vi "Create Property.vi"(8 "error in":errorcluster, 10 "Labview Type":T1, 11 "Description":string) -> (0 "error out":errorcluster, 3 "JSON Schema Property out":string)   [LabVIEW 2020, in "JSON Schema Generator.lvlib"]
uses:
  JSON Schema Generator.lvlib
  <vilib>/Utility/Data Type/Type Definitions/Data Type.ctl
  aea4ecb6-ee08-4fcf-bd9c-6a72ca557f06.vi
  1a4a9289-16be-4b5e-ac83-e746006c8e55.vi
  <vilib>/JDP Science/JSONtext/Variant to JSON Text.vi
  <vilib>/JDP Science/JSONtext/Get all Object Items.vi
  <vilib>/JDP Science/JSONtext/Set Multiple Object Items.vi
  <vilib>/JDP Science/JSONtext/LVClass Serializer/JSONtext LVClass Serializer.lvclass
  <vilib>/JDP Science/JSONtext/JSONtext.lvlib
  <vilib>/Utility/Data Type/NI_Data Type.lvlib
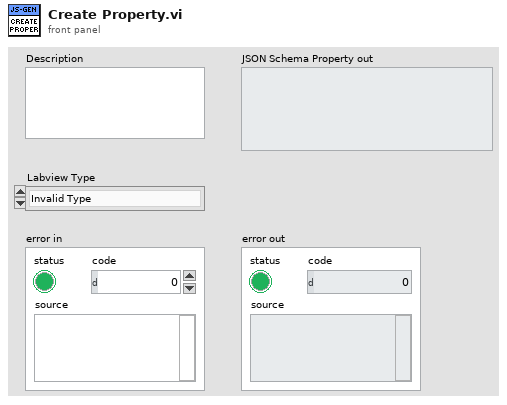
[diagram p1: front panel]
types:
  T1 = typedef "NI_Data Type.lvlib/Data Type.ctl" = enum8{"Invalid Type", "Void", "I8", "I16", "I32", "I64", "U8", "U16", "U32", "U64", "Single Float", "Double Float", "Extended Float", "Single Complex", "Double Complex", "Extended Complex", "Enum U8", "Enum U16", "Enum U32", "Enum U64", "Single Float With Unit", "Double Float With Unit", "Extended Float With Unit", "Single Complex with Unit", "Double Complex with Unit", "Extended Complex with Unit", "Boolean", "String", "Path", "Picture", "Tag", "Array", "Cluster", "Variant", "LV Variant", "Waveform", "Timestamp", "Digital Waveform", "Digital Data", "ExpressData", "Refnum", "External Data", "VI", "Poly VI", "LabVIEW Class Instance", "Fixed Point", "Set Collection", "Map Collection"}
  T2 = typedef "JSONtext.lvlib/JSON Value Type.ctl" = enum16{"Not a JSON Value", "JSON Object", "JSON Array", "String", "Number", "true", "false", "null"}
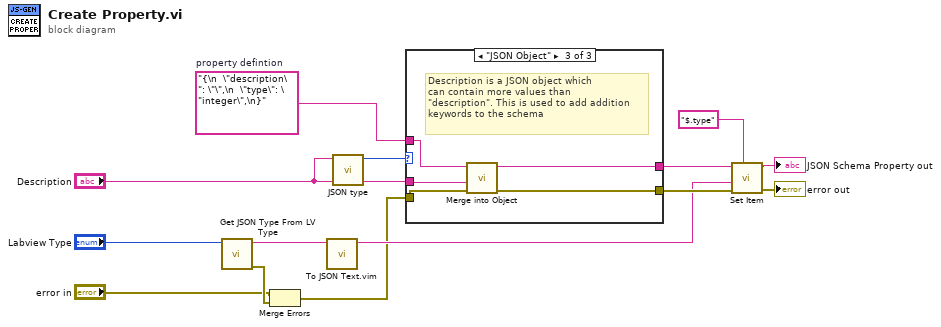
[diagram p0: block diagram]
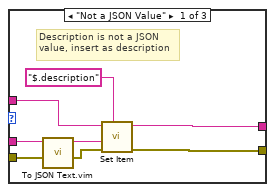
[diagram p2: hidden frame]
diagram:
  w11 = "{\n  \"description\": \"\",\n  \"type\": \"integer\",\n}"  # property defintion
  n1 = call "Get JSON Type From LV Type.vi"("Labview Datatype"="Labview Type") -> ("error out"=w13:errorcluster, "JSON Schema Type"=w5:string)  [unwired: 9 in]
  n2 = Merge Errors("error in", w13) -> (w4:errorcluster)
  n3 = call "To JSON Text.vim"("Anything"=w5) -> ("<JSON>"=w8:string)  [unwired: 9 in, 1 out]
  n4 = call <vilib>:"JSON type.vi"("JSON"="Description") -> ("JSON Value Type"=w1:T2)  [unwired: 9 in, 1 out]
  n5 = case shown="\"JSON Object\"" w1 {
    tunnel: [w22 w23 w28] -> w12
    tunnel: w11 -> [w21 w24 w26]
    tunnel: [w20 w24 w27] -> w9
    tunnel: w4 -> [w16 w23 w29]
    tunnel: "Description" -> [w19 _ w25]
    frame "Not a JSON Value" {
      # "Description is not a JSON\nvalue, insert as description"
      n6 = call "To JSON Text.vim"("error in (no error)"=w16, "Anything"=w19) -> ("error out"=w15:errorcluster, "<JSON>"=w17:string)  [unwired: 8 in]
      n7 = call <vilib>:"Set Item.vi"("$Path or Item Name"="$.description", "error in (no error)"=w15, "JSON to Insert"=w17, "JSON"=w21) -> ("error out"=w22:errorcluster, "<JSON>"=w20:string)  [unwired: 4 in, 1 out]
    }
    frame Default {
    }
    frame "JSON Object" {
      # "Description is a JSON object which\ncan contain more values than \n\"description\". This is used to add addition\nkeywords to the schema"
      n8 = call <vilib>:"Merge into Object.vi"("error in (no error)"=w29, "JSON Object to Merge"=w25, "JSON"=w26) -> ("error out"=w28:errorcluster, "<JSON>"=w27:string)  [unwired: 6 in]
    }
  }
  n9 = call <vilib>:"Set Item.vi"("$Path or Item Name"="$.type", "error in (no error)"=w12, "JSON to Insert"=w8, "JSON"=w9) -> ("error out"=→"error out":errorcluster, "<JSON>"=→"JSON Schema Property out":string)  [unwired: 4 in, 1 out]
